vi "WLAN Configure SEM.vi"(0 "Instrument Handle In":refnum<k21>, 1 "Selector String":string, 5 "WLAN SEM Configuration":T1={"Sweep Time Auto"=1, "Sweep Time (s)"=0.001, "Span Auto"=1, "Span (Hz)"=100000000.0, "Averaging Enabled"=0, "Averaging Count"=5, "Averaging Type"=0} {"Averaging Type" items=["RMS", "Log", "Scalar", "Max", "Min"]; "Averaging Enabled" items=["False", "True"]; "Span (Hz)" format="%.3p"; "Span Auto" items=["False", "True"]; "Sweep Time (s)" format="%.3p"; "Sweep Time Auto" items=["False", "True"]}, 11 "error in (no error)":errorcluster) -> (4 "Instrument Handle Out":refnum<k21>, 15 "error out":errorcluster)   [LabVIEW 2016, in "RFmxWLAN.lvlib"]
doc: "Configures common settings for the SEM measurement and selects the measurement."
uses:
  RFmxWLAN.lvlib
  Typedefs/WLAN SEM Configuration.ctl
  <vilib>/RFmx/WLAN/mx/RFmxWLAN.llb/RFmxWLAN Select Measurement (Single).vi
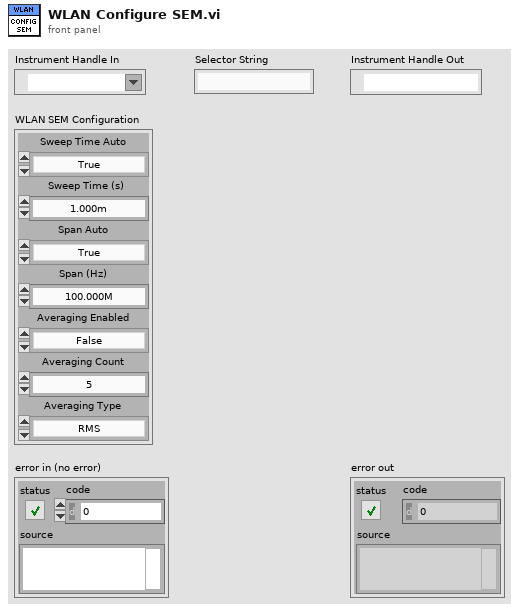
[diagram p1: front panel]
types:
  T1 = typedef "RFmxWLAN.lvlib/WLAN SEM Configuration.ctl" = cluster{"Sweep Time Auto":i32, "Sweep Time (s)":dbl, "Span Auto":i32, "Span (Hz)":dbl, "Averaging Enabled":i32, "Averaging Count":i32, "Averaging Type":i32}
  T2 = enum16{"TXP", "PowerRamp", "DSSSModAcc", "OFDMModAcc", "SEM"}
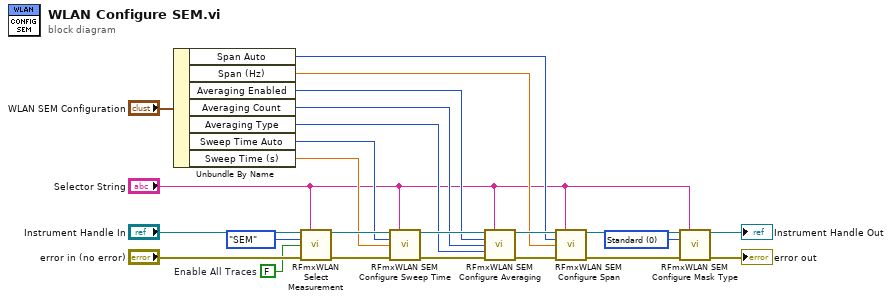
[diagram p0: block diagram]
diagram:
  w1 = FALSE  # Enable All Traces
  w7 = 0 items=["Standard", "Custom"] ("Mask Type")
  n1 = Unbundle By Name("WLAN SEM Configuration") -> ("Span Auto"=w6:i32, "Span (Hz)"=w5:dbl, "Averaging Enabled"=w8:i32, "Averaging Count"=w9:i32, "Averaging Type"=w10:i32, "Sweep Time Auto"=w12:i32, "Sweep Time (s)"=w11:dbl)
  n2 = call-poly <vilib>:"RFmxWLAN Select Measurement.vi"("Instrument Handle In"="Instrument Handle In", "Selector String"="Selector String", "Measurement"=T2."SEM", "Enable All Traces"=w1, "error in (no error)"="error in (no error)") -> ("Instrument Handle Out"=w17:refnum<k21>, "error out"=w21:errorcluster)  [unwired: 9 in]
  n3 = call <vilib>:"RFmxWLAN SEM Configure Sweep Time.vi"("Instrument Handle In"=w17, "Selector String"="Selector String", "Sweep Time Auto"=w12, "Sweep Time Interval (s)"=w11, "error in (no error)"=w21) -> ("Instrument Handle Out"=w18:refnum<k21>, "error out"=w19:errorcluster)  [unwired: 9 in]
  n4 = call <vilib>:"RFmxWLAN SEM Configure Averaging.vi"("Instrument Handle In"=w18, "Selector String"="Selector String", "Averaging Enabled"=w8, "Averaging Count"=w9, "Averaging Type"=w10, "error in (no error)"=w19) -> ("Instrument Handle Out"=w15:refnum<k21>, "error out"=w22:errorcluster)  [unwired: 8 in]
  n5 = call <vilib>:"RFmxWLAN SEM Configure Span.vi"("Instrument Handle In"=w15, "Selector String"="Selector String", "Span Auto"=w6, "Span (Hz)"=w5, "error in (no error)"=w22) -> ("Instrument Handle Out"=w14:refnum<k21>, "error out"=w16:errorcluster)  [unwired: 9 in]
  n6 = call <vilib>:"RFmxWLAN SEM Configure Mask Type.vi"("Instrument Handle In"=w14, "Selector String"="Selector String", "Mask Type"=w7, "error in (no error)"=w16) -> ("Instrument Handle Out"=→"Instrument Handle Out":refnum<k21>, "error out"=→"error out":errorcluster)  [unwired: 10 in]
